vi "Read FXP.vi"(7 "FXP Configuration":T1, 8 "error in":errorcluster, 9 "RegisterOffset":u32, 10 "register name":string, 11 "session in":u32) -> (0 "error out":errorcluster, 2 "DBL Value":dbl, 3 "session out":u32)   [LabVIEW 2020, in "FPGA Register IO.lvlib"]
uses:
  FPGA Register IO.lvlib
  TypeDefs/FXP Configuration.ctl
  <vilib>/fxp/LVFixedPointRepBitsTypeDef.ctl
  <vilib>/fxp/LVFixedPointRepRangeTypeDef.ctl
  Error Handling/Error 6003.vi
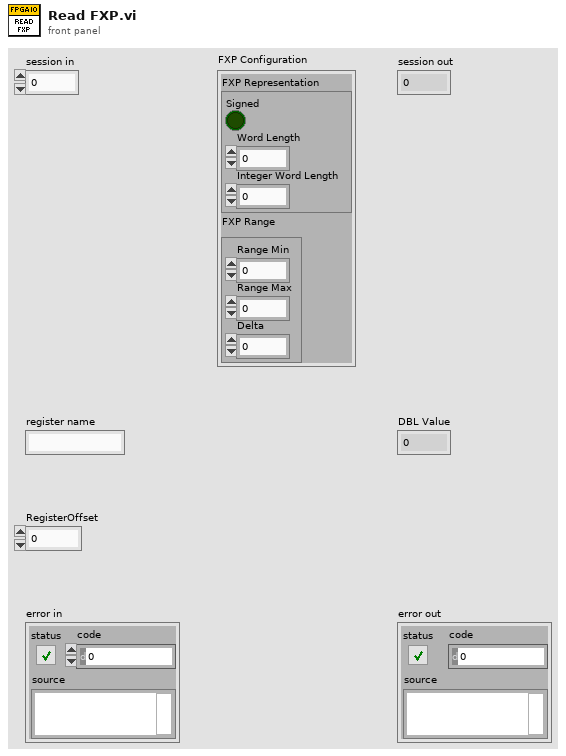
[diagram p1: front panel]
types:
  T1 = typedef "FPGA Register IO.lvlib/FXP Configuration.ctl" = cluster{"FXP Representation":T2, "FXP Range":T3}
  T2 = typedef "LVFixedPointRepBitsTypeDef.ctl" = cluster{"Signed":bool, "Word Length":u32, "Integer Word Length":i32}
  T3 = typedef "LVFixedPointRepRangeTypeDef.ctl" = cluster{"Range Min":dbl, "Range Max":dbl, "Delta":dbl}
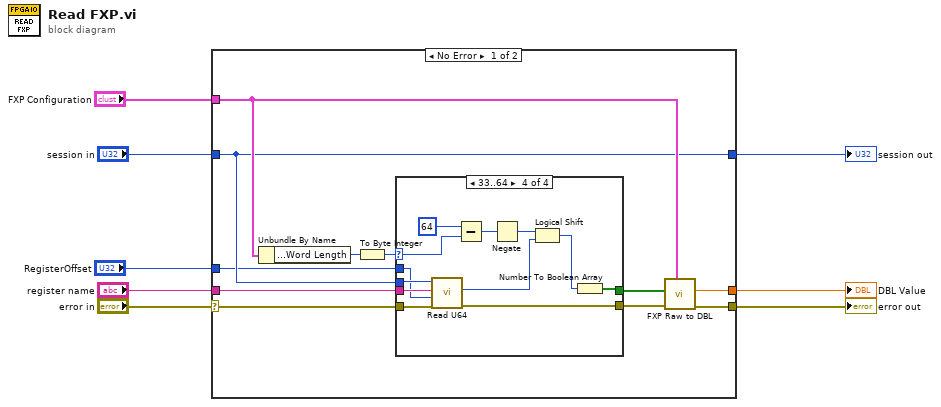
[diagram p0: block diagram]
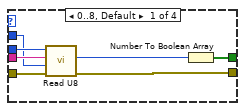
[diagram p2: hidden frame]
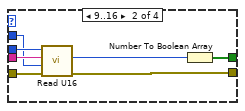
[diagram p3: hidden frame]
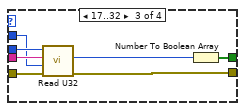
[diagram p4: hidden frame]
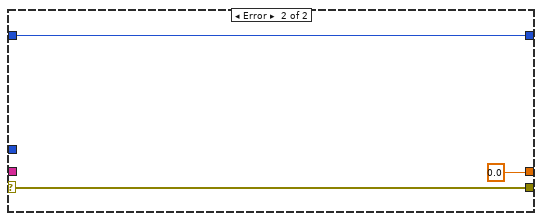
[diagram p5: hidden frame]
diagram:
  n1 = case shown="No Error" "error in" {
    selector: "error in" -> [w12 w55]
    tunnel: "session in" -> [w14 w54]
    tunnel: [w19 w55] -> w8
    tunnel: "register name" -> [w17 _]
    tunnel: [w14 w54] -> w7
    tunnel: [w18 0.0 ("DBL Value")] -> w6
    tunnel: "FXP Configuration" -> [w15 _]
    tunnel: "RegisterOffset" -> [w9 _]
    frame No Error {
      n2 = Unbundle By Name(w15) -> ("FXP Representation.Word Length"=w16:u32)
      n3 = To Byte Integer(number=w16) -> (8bit integer=w10:i8)
      n4 = case shown="33..64" w10 {
        selector: w10 -> [_ _ _ w44]
        tunnel: w17 -> [w25 w31 w38 w50]
        tunnel: [w26 w29 w36 w49] -> w11
        tunnel: w14 -> [w24 w32 w39 w51]
        tunnel: [w23 w30 w37 w48] -> w13
        tunnel: w12 -> [w22 w33 w40 w52]
        tunnel: w9 -> [w21 w28 w35 w41]
        frame 0..8, Default {
          n5 = call "Read U8.vi"("error in"=w22, "RegisterOffset"=w21, "register name"=w25, "session in"=w24) -> ("error out"=w23:errorcluster, "value out"=w20:u8)  [unwired: 5 in, 1 out]
          n6 = Number To Boolean Array(number=w20) -> (Boolean array=w26:bool[])
        }
        frame 9..16 {
          n7 = call "Read U16.vi"("error in"=w33, "RegisterOffset"=w28, "register name"=w31, "session in"=w32) -> ("error out"=w30:errorcluster, "value out"=w27:u16)  [unwired: 5 in, 1 out]
          n8 = Number To Boolean Array(number=w27) -> (Boolean array=w29:bool[])
        }
        frame 17..32 {
          n9 = call "Read U32.vi"("error in"=w40, "RegisterOffset"=w35, "register name"=w38, "session in"=w39) -> ("error out"=w37:errorcluster, "value out"=w34:u32)  [unwired: 5 in, 1 out]
          n10 = Number To Boolean Array(number=w34) -> (Boolean array=w36:bool[])
        }
        frame 33..64 {
          n11 = call "Read U64.vi"("error in"=w52, "RegisterOffset"=w41, "register name"=w50, "session in"=w51) -> ("error out"=w48:errorcluster, "value out"=w43:u64)  [unwired: 5 in, 1 out]
          n12 = Subtract(x=i8 64 ("y"), y=w44) -> (x-y=w46:i8)
          n13 = Negate(x=w46) -> (-x=w45:i8)
          n14 = Logical Shift(y=w45, x=w43) -> (x << y=w42:u64)
          n15 = Number To Boolean Array(number=w42) -> (Boolean array=w49:bool[])
        }
      }
      n16 = call "FXP Raw to DBL.vi"("FXP Configuration"=w15, "error in (no error)"=w13, "Bool Data"=w11) -> ("error out"=w19:errorcluster, "DBL Value"=w18:dbl)  [unwired: 7 in]
    }
    frame Error {
    }
  }
  "error out" <- w8
  "session out" <- w7
  "DBL Value" <- w6
